vi "Initialize.vi"(8 "error in (no error)":errorcluster, 10 "parent":string, 11 "string handler":refnum<class "String Handler.lvclass">) -> (0 "error out":errorcluster, 2 "name":string, 3 "dup string handler":refnum<class "String Handler.lvclass">)   [LabVIEW 2018, in "GLog.lvlib" / "String Handler.lvclass"]
uses:
  String Handler.lvclass
  String Handler.lvclass/String Handler.ctl
  extension/formatting_handler_interface/Formatting Handler.lvclass
  UI Updater/UI Updater.lvlib
panel:
  # "Connector Pane"
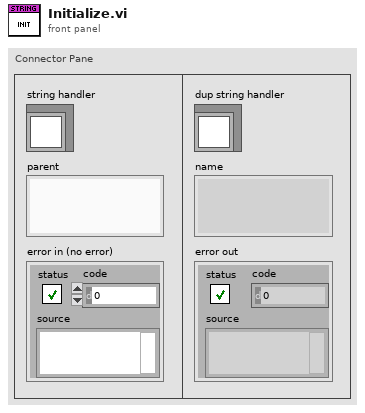
[diagram p1: front panel]
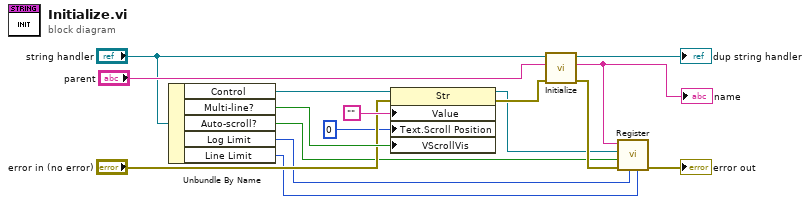
[diagram p0: block diagram]
diagram:
  n1 = Unbundle By Name("string handler") -> ("Control"=w16:refnum<vi>, "Multi-line?"=w14:bool, "Auto-scroll?"=w1:bool, "Log Limit"=w3:u32, "Line Limit"=w2:u32)
  n2 = property class="Str"(reference=w16, error in="error in (no error)", "Value"="", "Text.Scroll Position"=u32 0, "VScrollVis"=w14) -> (reference out=w5:refnum<vi>, error out=w11:errorcluster)
  n3 = call-parent "Initialize.vi"("error in (no error)"=w11, "logger name"="parent", "handler in"="string handler") -> ("error out"=w7:errorcluster, "handler name"=w4:string, "handler out"=→"dup string handler":refnum<class "String Handler.lvclass">)  [unwired: 6 in]
  "name" <- w4
  n4 = call "Register.vi"("line limit"=w2, "log limit"=w3, "error in (no error)"=w7, "auto-scroll"=w1, "ctl ref"=w5, "handler name"=w4) -> ("error out"=→"error out":errorcluster)  [unwired: 5 in]
